vi "Init.vi"(8 "error in (no error)":errorcluster, 10 "Image Refnum":refnum<vi>, 11 "ImageHandler:Varex-ImageHandler in":refnum<class "Varex-ImageHandler.lvclass">) -> (0 "error out":errorcluster, 3 "ImageHandler:Varex-ImageHandler out":refnum<class "Varex-ImageHandler.lvclass">)   [LabVIEW 2022 SP3, in "ImageHandler.lvlib" / "Varex-ImageHandler.lvclass"]
uses:
  Varex-ImageHandler.lvclass
  Varex-ImageHandler.lvclass/Varex-ImageHandler.ctl
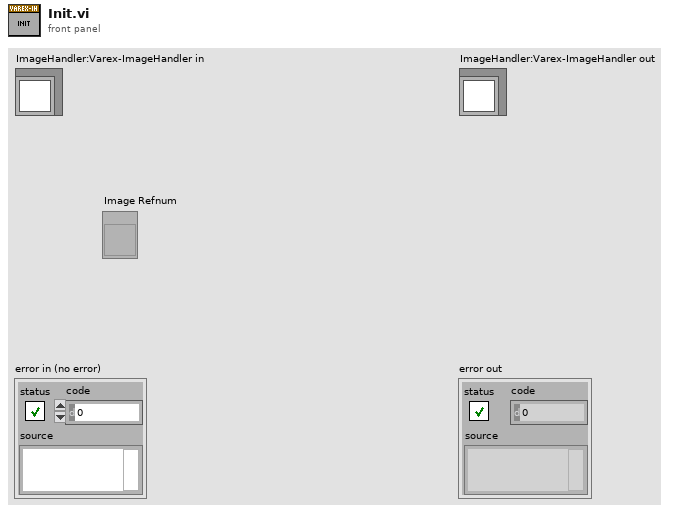
[diagram p1: front panel]
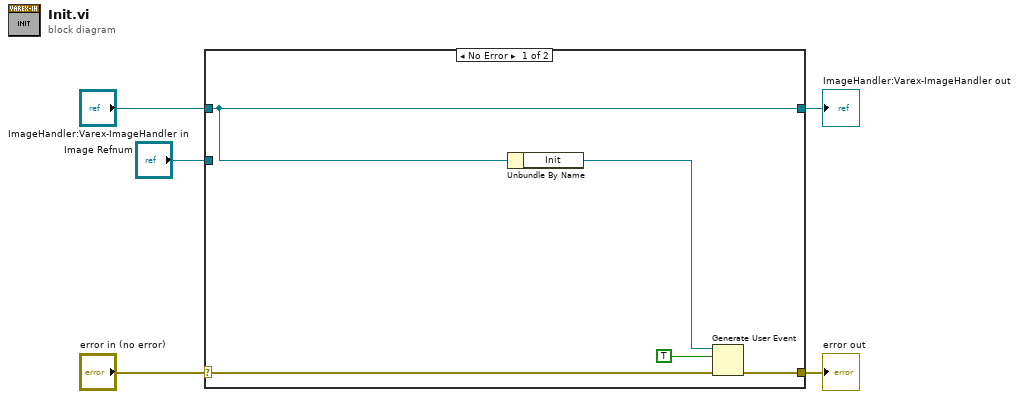
[diagram p0: block diagram]
diagram:
  n1 = case shown="No Error" "error in (no error)" {
    selector: "error in (no error)" -> [w10 w12]
    tunnel: [w8 w12] -> w4
    tunnel: [w9 w11] -> w2
    tunnel: "ImageHandler:Varex-ImageHandler in" -> [w9 w11]
    tunnel: "Image Refnum" -> [_ _]
    frame No Error {
      n2 = Unbundle By Name(w9) -> ("Init"=w7:refnum<user-event>)
      n3 = Generate User Event(user event=w7, event data cluster=TRUE ("event data"), error in=w10) -> (error out=w8:errorcluster)  [unwired: 1 in, 1 out]
    }
    frame Error {
    }
  }
  "error out" <- w4
  "ImageHandler:Varex-ImageHandler out" <- w2
